vi "SplineHelp_getQuinticSplinesFromControlVectors.vi"(11 "ControlVectors":T1[](array[typedef])) -> (0 "error out":errorcluster, 3 "splines":T2[](array[typedef]))   [LabVIEW 2019, in "Trajectory_Library.lvlib"]
doc: "Returns a set of quintic splines corresponding to the provided control vectors. The user is free to set the direction of all control vectors. Continuous curvature is guaranteed throughout the path.\n\nParameters:\n - controlVectors - The control vectors.\n\nReturns:\n - Splines - A vector of quintic hermite splines that interpolate through the provided waypoints.\n - Error Out - The returned error cluster"
uses:
  Trajectory_Library.lvlib
  TypeDef/SPLINE_CTRL_VECTOR.ctl
  <vilib>/Analysis/Matrix/Datatypes/RealMatrix.ctl
  <vilib>/Analysis/Matrix/NI_Matrix.lvlib
  TypeDef/SPLINE.ctl
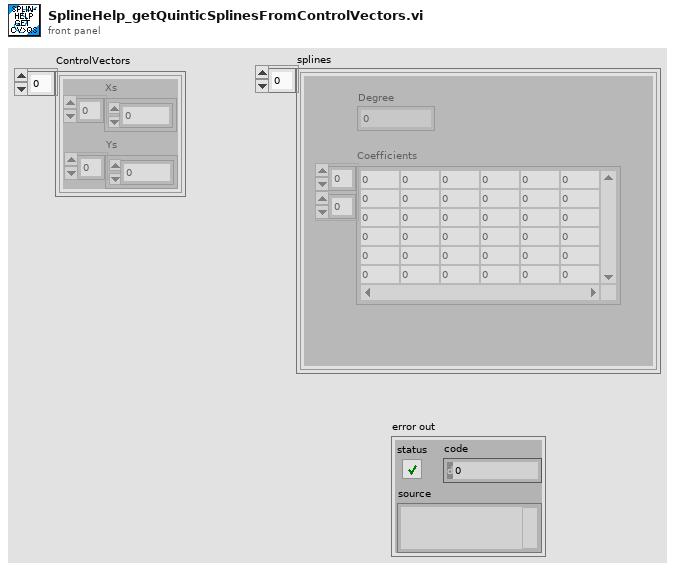
[diagram p1: front panel]
types:
  T1 = typedef "Trajectory_Library.lvlib/SPLINE_CTRL_VECTOR.ctl" = cluster{"Xs":dbl[], "Ys":dbl[]}
  T2 = typedef "Trajectory_Library.lvlib/SPLINE.ctl" = cluster{"Degree":i32, "Coefficients":T3}
  T3 = typedef "NI_Matrix.lvlib/RealMatrix.ctl" = dbl[][]
  T4 = typedef "WPILib_Math.lvlib/SPLINE.ctl" = cluster{"Degree":i32, "Coefficients":T3}
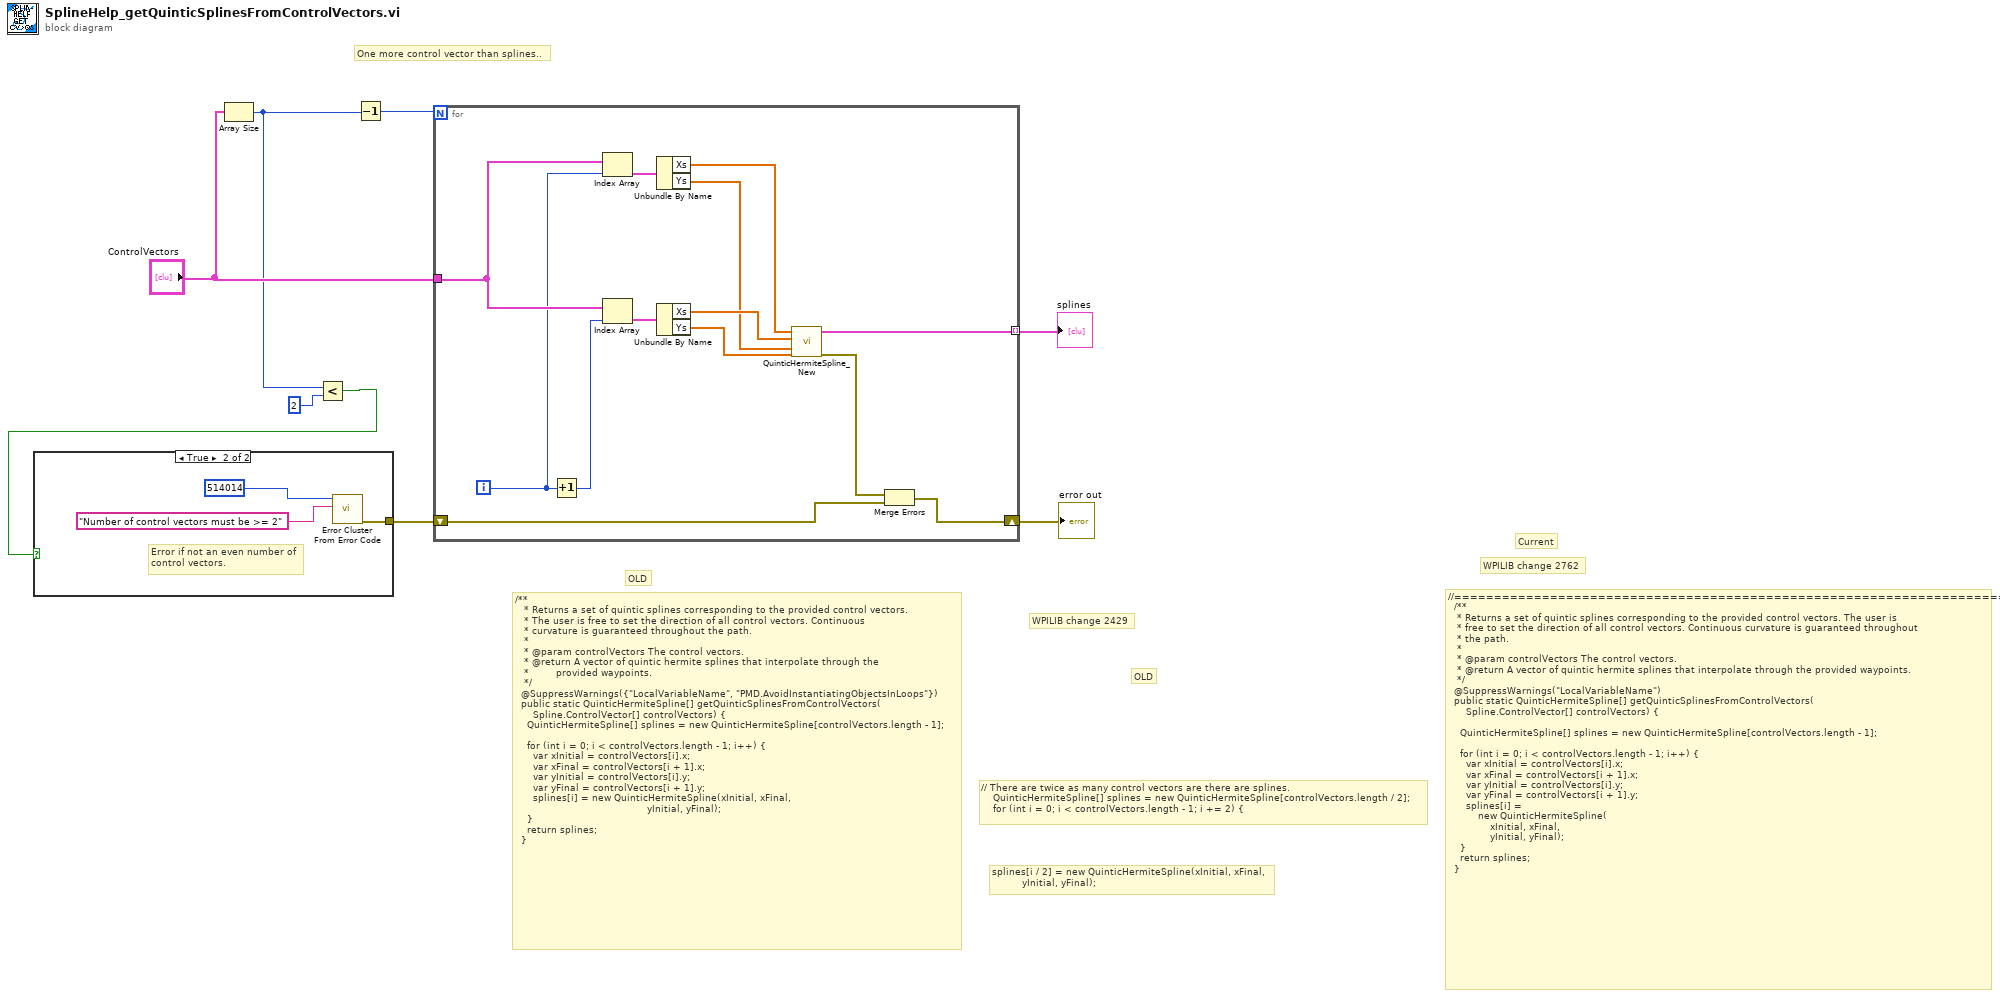
[diagram p0: block diagram]
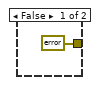
[diagram p2: hidden frame]
diagram:
  # "Current"
  # "OLD"
  # "OLD"
  # "One more control vector than splines.."
  # "//======================================================================\n  /**\n   * Returns a set of quintic splines corresponding to the provided control vectors. The user is\n   * free to set the direction of all control vectors. Continuous curvature is guaranteed throughout\n   * the path.\n   *\n   * @param controlVectors The control vectors.\n   * @return A vector of quintic hermite splines that interpolate through the provided waypoints.\n   */\n  @SuppressWarnings(\"LocalVariableName\")\n  public static QuinticHermiteSpline[] getQuinticSplinesFromControlVectors(\n      Spline.ControlVector[] controlVectors) {\n\n    QuinticHermiteSpline[] splines = new QuinticHermiteSpline[controlVectors.length - 1];\n\n    for (int i = 0; i < controlVectors.length - 1; i++) {\n      var xInitial = controlVectors[i].x;\n      var xFinal = controlVectors[i + 1].x;\n      var yInitial = controlVectors[i].y;\n      var yFinal = controlVectors[i + 1].y;\n      splines[i] =\n          new QuinticHermiteSpline(\n              xInitial, xFinal,\n              yInitial, yFinal);\n    }\n    return splines;\n  }"
  # "WPILIB change 2762"
  # "splines[i / 2] = new QuinticHermiteSpline(xInitial, xFinal,\n          yInitial, yFinal);"
  # "WPILIB change 2429"
  # "// There are twice as many control vectors are there are splines.\n    QuinticHermiteSpline[] splines = new QuinticHermiteSpline[controlVectors.length / 2];\n    for (int i = 0; i < controlVectors.length - 1; i += 2) {"
  # "/**\n   * Returns a set of quintic splines corresponding to the provided control vectors.\n   * The user is free to set the direction of all control vectors. Continuous\n   * curvature is guaranteed throughout the path.\n   *\n   * @param controlVectors The control vectors.\n   * @return A vector of quintic hermite splines that interpolate through the\n   *         provided waypoints.\n   */\n  @SuppressWarnings({\"LocalVariableName\", \"PMD.AvoidInstantiatingObjectsInLoops\"})\n  public static QuinticHermiteSpline[] getQuinticSplinesFromControlVectors(\n      Spline.ControlVector[] controlVectors) {\n    QuinticHermiteSpline[] splines = new QuinticHermiteSpline[controlVectors.length - 1];\n\n    for (int i = 0; i < controlVectors.length - 1; i++) {\n      var xInitial = controlVectors[i].x;\n      var xFinal = controlVectors[i + 1].x;\n      var yInitial = controlVectors[i].y;\n      var yFinal = controlVectors[i + 1].y;\n      splines[i] = new QuinticHermiteSpline(xInitial, xFinal,\n                                            yInitial, yFinal);\n    }\n    return splines;\n  }"
  n1 = Array Size(array="ControlVectors") -> (size(s)=w2:i32)
  n2 = Less?(x=w2, y=2) -> (x < y?=w4:bool)
  n3 = case shown="True" w4 {
    tunnel: [errorcluster {"status"=FALSE, "code"=0, "source"=""} ("error out") w10] -> w5
    frame False {
    }
    frame True {
      # "Error if not an even number of\ncontrol vectors."
      n4 = call <vilib>:"Error Cluster From Error Code.vi"("error message (\"\")"="Number of control vectors must be >= 2" ("error message (\"\")"), "error code (0)"=514014) -> ("error out"=w10:errorcluster)  [unwired: 7 in]
    }
  }
  n5 = Decrement(x=w2) -> (x-1=w1:i32)
  n6 = for {
    N: w1 -> [_]
    tunnel: [w25] -> w8 mode=indexing
    shift-right: [w22] -> w7
    shift-left: w5 -> [w23]
    tunnel: "ControlVectors" -> [w20]
    i -> [w13]
    n7 = Increment(x=w13) -> (x+1=w24:i32)
    n8 = Index Array(array=w20, index=w13) -> (element=w19:T1)
    n9 = Index Array(array=w20, index=w24) -> (element=w18:T1)
    n10 = Unbundle By Name(w19) -> ("Xs"=w17:dbl[], "Ys"=w15:dbl[])
    n11 = Unbundle By Name(w18) -> ("Xs"=w16:dbl[], "Ys"=w14:dbl[])
    n12 = call "QuinticHermiteSpline_New.vi"("yFinalCtrlVector"=w14, "yInitialCtrlVector"=w15, "xFinalCtrlVector"=w16, "XInitialCtrlVector"=w17) -> ("error out"=w21:errorcluster, "QuinticHermiteSpline"=w25:T4)  [unwired: 6 in]
    n13 = Merge Errors(w21, w23) -> (w22:errorcluster)
  }
  "error out" <- w7
  "splines" <- w8
